vi "GetElement(Single).vi"(7 "Qualified Name":string, 8 "error in (no error)":errorcluster, 10 "Key":string, 11 "ConfigManager.Text in":refnum<class "ConfigManager.Text.lvclass">) -> (0 "error out":errorcluster, 1 "Value":string, 2 "Key":string, 3 "ConfigManager.Text out":refnum<class "ConfigManager.Text.lvclass">, 4 "found":bool)   [LabVIEW 2013, in "CfgManager.Text.lvlib" / "ConfigManager.Text.lvclass"]
uses:
  ConfigManager.Text.lvclass
  Query -- cluster.ctl
  Response - cluster.ctl
  ConfigManager.Text.lvclass/ConfigManager.Text.ctl
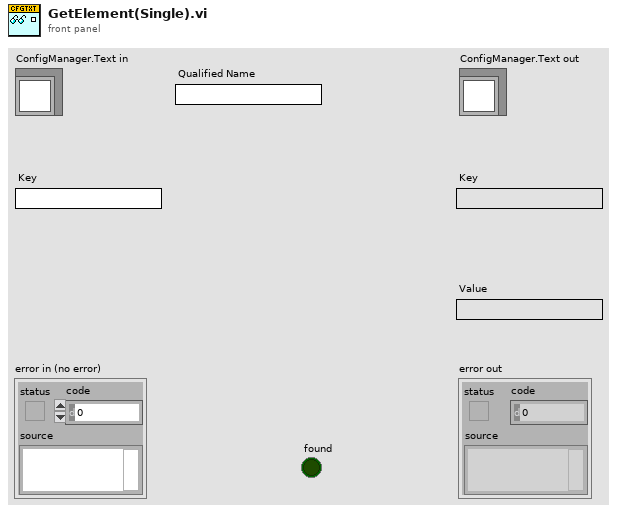
[diagram p1: front panel]
types:
  T1 = typedef "CfgManager.Text.lvlib/ConfigManager.Text.lvclass/Response - cluster.ctl" = cluster{"Section":string[], "Keys":string[], "Values":string[], "Found":bool[]}
  T2 = typedef "CfgManager.Text.lvlib/ConfigManager.Text.lvclass/Query -- cluster.ctl" = cluster{"Qualified Name":string[], "Keys":string[]}
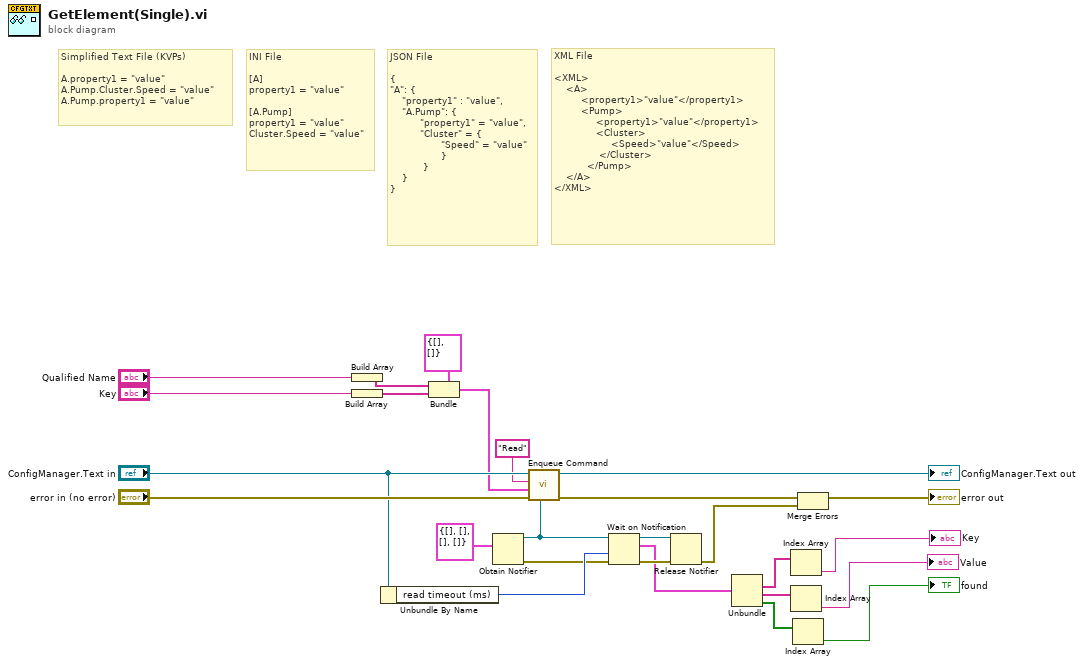
[diagram p0: block diagram]
diagram:
  # "XML File\n\n<XML>\n    <A>\n         <property1>\"value\"</property1>\n         <Pump> \n              <property1>\"value\"</property1>\n              <Cluster>\n                   <Speed>\"value\"</Speed>\n               </Cluster>  \n           </Pump>\n    </A>\n</XML>"
  # "JSON File\n\n{\n\"A\": {\n    \"property1\" : \"value\",\n    \"A.Pump\": {\n          \"property1\" = \"value\",\n          \"Cluster\" = {\n                 \"Speed\" = \"value\"\n                 }\n           }\n    }\n}"
  # "INI File\n\n[A]\nproperty1 = \"value\"\n\n[A.Pump]\nproperty1 = \"value\"\nCluster.Speed = \"value\""
  # "Simplified Text File (KVPs)\n\nA.property1 = \"value\"\nA.Pump.Cluster.Speed = \"value\"\nA.Pump.property1 = \"value\""
  n1 = Build Array("Qualified Name") -> (w6:string[])
  n2 = Build Array("Key") -> (w10:string[])
  n3 = Unbundle By Name("ConfigManager.Text in") -> ("read timeout (ms)"=w14:i32)
  n4 = Bundle(cluster=T2 {"Qualified Name"=[], "Keys"=[]} ("Query"), "Qualified Name"=w6, "Keys"=w10) -> (w8:T2)
  n5 = Obtain Notifier(notification data type=T1 {"Section"=[], "Keys"=[], "Values"=[], "Found"=[]} ("response")) -> (notifier out=w7:refnum<notifier>, error out=w13:errorcluster)  [unwired: 3 in, 1 out]
  n6 = call "Enqueue Command.vi"("query notifier"=w7, "error in (no error)"="error in (no error)", "args"=w8, "command"="Read", "ConfigManager.Text in"="ConfigManager.Text in") -> ("error out"=w3:errorcluster, "ConfigManager.Text out"=→"ConfigManager.Text out":refnum<class "ConfigManager.Text.lvclass">)  [unwired: 4 in, 1 out]
  n7 = Wait on Notification(notifier=w7, timeout in ms (-1)=w14, error in (no error)=w13) -> (notifier out=w16:refnum<notifier>, notification=w11:T1, error out=w15:errorcluster)  [unwired: 1 in, 1 out]
  n8 = Release Notifier(notifier=w16, error in (no error)=w15) -> (error out=w12:errorcluster)  [unwired: 1 in, 2 out]
  n9 = Unbundle(w11) -> ("Keys"=w2:string[], "Values"=w4:string[], "Found"=w5:bool[])  [unwired: 1 out]
  n10 = Index Array(array=w2) -> (element=→"Key":string)  [unwired: 1 in]
  n11 = Index Array(array=w4) -> (element=→"Value":string)  [unwired: 1 in]
  n12 = Index Array(array=w5) -> (element=→"found":bool)  [unwired: 1 in]
  n13 = Merge Errors(w3, w12) -> (→"error out":errorcluster)
